vi "Arduino Writter.vi"() -> ()   [LabVIEW 2013]
uses:
  <vilib>/Instr/_visa.llb/VISA Configure Serial Port (Instr).vi
panel:
  in  "Baud Rate":u32=9600
  in  "COM Port":refnum<visa-resource-name>="COM8"
  out "Debug - Return from Arduino":string
  in  "Connect":bool
  in  "Stop Button":bool
  in  "Gain":dbl min=0.0 step=0.001 format="%.3f"
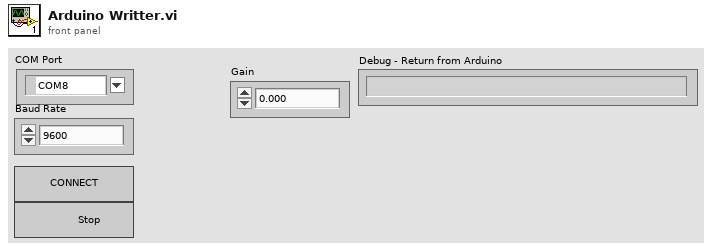
[diagram p1: front panel]
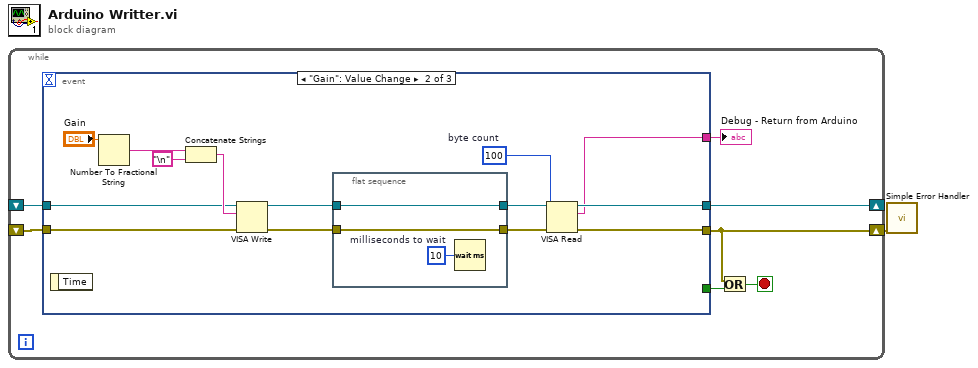
[diagram p0: block diagram]
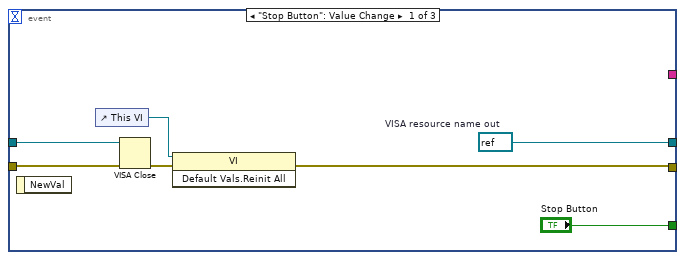
[diagram p2: hidden frame]
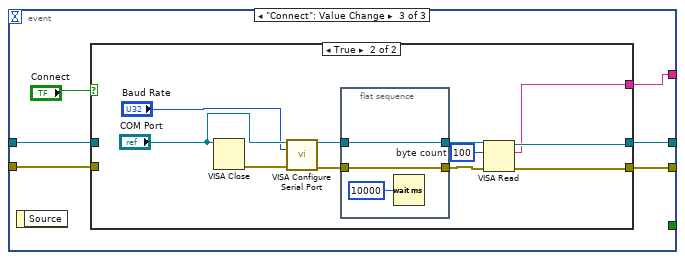
[diagram p3: hidden frame]
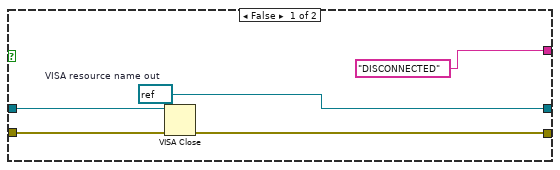
[diagram p4: hidden frame]
diagram:
  n1 = while {
    shift-right: [w2] -> w1
    shift-left: _ -> [w5]
    shift-right: [w7] -> _
    shift-left: _ -> [w6]
    stop <- w3 stop-if-true
    n2 = event shown="[1] \"Gain\": Value Change" {
      selector: _ -> [_ _ _]
      dyn-events: _ -> [_ _ _]
      timeout: _ -> [_ _ _]
      tunnel: ["Stop Button" _ _] -> w8
      tunnel: [w12 w22 w37] -> w7
      tunnel: [w9 w23 w36] -> w2
      tunnel: w6 -> [w14 w25 w35]
      tunnel: w5 -> [w13 w24 w34]
      tunnel: [_ w16 w33] -> w4
      event "Stop Button": Value Change {
        w12 = refnum<visa-resource-name> refnum  # VISA resource name out
        n3 = event-data() -> ()  [unwired: 1 in, 1 out]
        n4 = control-ref of="This VI"() -> (w11:refnum<vi>)
        n5 = VISA Close(VISA resource name=w14, error in (no error)=w13) -> (error out=w10:errorcluster)
        n6 = invoke class="VI" method="Default Vals.Reinit All"(reference=w11, error in=w10) -> (error out=w9:errorcluster)  [unwired: 1 in, 2 out]
      }
      event "Gain": Value Change {
        w19 = u32 100  # byte count
        n7 = event-data() -> ()  [unwired: 1 in, 1 out]
        n8 = Number To Fractional String(number="Gain") -> (F-format string=w27:string)  [unwired: 3 in]
        n9 = Concatenate Strings(w27, "\n") -> (w28:string)
        n10 = VISA Write(VISA resource name=w25, write buffer=w28, error in (no error)=w24) -> (VISA resource name out=w21:refnum<visa-resource-name>, error out=w18:errorcluster)  [unwired: 1 out]
        n11 = flat-sequence {
          tunnel: w21 -> [w32]
          tunnel: [w32] -> w20
          tunnel: w18 -> [w31]
          tunnel: [w31] -> w17
          frame #0 {
            w30 = u32 10  # milliseconds to wait
            n12 = Wait (ms)(milliseconds to wait=w30) -> ()  [unwired: 1 out]
          }
        }
        n13 = VISA Read(VISA resource name=w20, byte count=w19, error in (no error)=w17) -> (VISA resource name out=w22:refnum<visa-resource-name>, read buffer=w16:string, error out=w23:errorcluster)  [unwired: 1 out]
      }
      event "Connect": Value Change {
        n14 = event-data() -> ()  [unwired: 1 in, 1 out]
        n15 = case shown="True" "Connect" {
          tunnel: [w40 w47] -> w37
          tunnel: [w42 w46] -> w36
          tunnel: w35 -> [w43 _]
          tunnel: w34 -> [w41 _]
          tunnel: ["DISCONNECTED" ("read buffer") w44] -> w33
          frame False {
            w40 = refnum<visa-resource-name> refnum  # VISA resource name out
            n16 = VISA Close(VISA resource name=w43, error in (no error)=w41) -> (error out=w42:errorcluster)
          }
          frame True {
            w45 = u32 100  # byte count
            n17 = VISA Close(VISA resource name="COM Port") -> (error out=w54:errorcluster)  [unwired: 1 in]
            n18 = call-poly "VISA Configure Serial Port"("VISA resource name"="COM Port", "baud rate (9600)"="Baud Rate", "error in (no error)"=w54) -> ("VISA resource name out"=w53:refnum<visa-resource-name>, "error out"=w52:errorcluster)  [unwired: 11 in]
            n19 = flat-sequence {
              tunnel: w53 -> [w55]
              tunnel: w52 -> [w56]
              tunnel: [w56] -> w48
              tunnel: [w55] -> w49
              frame #0 {
                n20 = Wait (ms)(milliseconds to wait=u32 10000) -> ()  [unwired: 1 out]
              }
            }
            n21 = VISA Read(VISA resource name=w49, byte count=w45, error in (no error)=w48) -> (VISA resource name out=w47:refnum<visa-resource-name>, read buffer=w44:string, error out=w46:errorcluster)  [unwired: 1 out]
          }
        }
      }
    }
    "Debug - Return from Arduino" <- w4
    n22 = Or(x=w2, y=w8) -> (x .or. y?=w3:bool)
  }
  n23 = call <vilib>:"Simple Error Handler.vi"("error in (no error)"=w1) -> ()  [unwired: 4 in, 5 out]
